vi "Stop All Helper Loops.vi"(8 "error in (no error)":errorcluster) -> (0 "error out":errorcluster)   [LabVIEW 2020, in "Helper Loop.lvclass"]
doc: "すべてのヘルパーループを終了し、リソースを破棄します。"
uses:
  Helper Loop.lvclass
  Helper Loop.lvclass/Helper Loop.ctl
  Sub/Helper Loop Map FGV Action.ctl
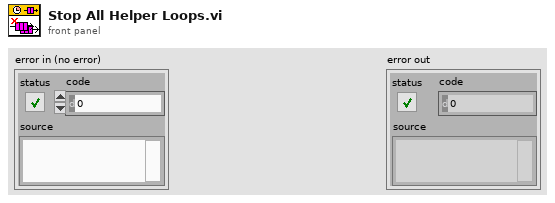
[diagram p1: front panel]
types:
  T1 = typedef "Helper Loop.lvclass/Helper Loop Map FGV Action.ctl" = enum16{"Get Pausing Helper Loop", "Register Active Helper Loop", "Pause Helper Loop", "Close Helper Loop", "Get All Helper Loops"}
  T2 = cluster{"Helper Loop Out":refnum<class "Helper Loop.lvclass">, "VI Reference":refnum<vi>}[]
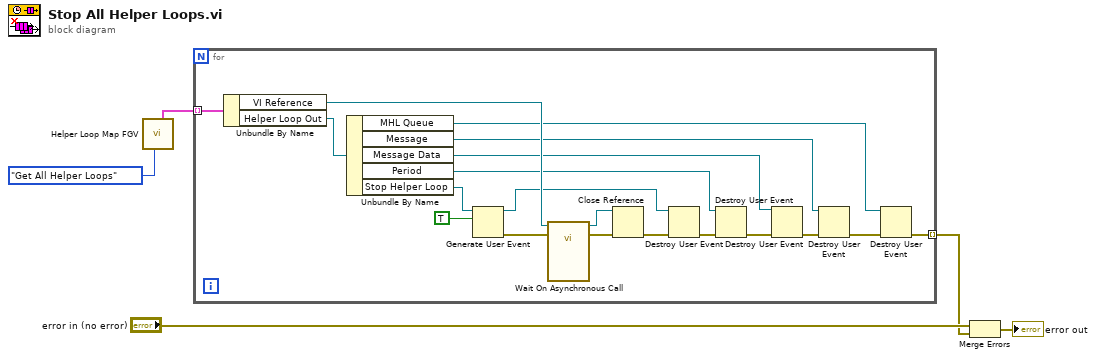
[diagram p0: block diagram]
diagram:
  n1 = call "Helper Loop Map FGV.vi"("Action"=Helper_Loop_Map_FGV_Action."Get All Helper Loops") -> ("All Helper Queues"=w4:T2)  [unwired: 7 in, 3 out]
  n2 = for {
    tunnel: w4 -> [w24] mode=indexing
    tunnel: [w6] -> w1 mode=indexing
    n3 = Unbundle By Name(w24) -> ("VI Reference"=w19:refnum<vi>, "Helper Loop Out"=w23:refnum<class "Helper Loop.lvclass">)
    n4 = Unbundle By Name(w23) -> ("MHL Queue"=w7:refnum<user-event>, "Message"=w8:refnum<user-event>, "Message Data"=w9:refnum<user-event>, "Period"=w10:refnum<user-event>, "Stop Helper Loop"=w22:refnum<user-event>)
    n5 = Generate User Event(user event=w22, event data cluster=TRUE ("event data")) -> (user event out=w15:refnum<user-event>, error out=w20:errorcluster)  [unwired: 2 in]
    n6 = call-by-ref "Wait On Asynchronous Call"(reference=w19, error in=w20) -> (reference out=w17:refnum<vi>, error out=w18:errorcluster)  [unwired: 11 in, 1 out]
    n7 = Close Reference(reference=w17, error in (no error)=w18) -> (error out=w16:errorcluster)
    n8 = Destroy User Event(user event=w15, error in=w16) -> (error out=w14:errorcluster)
    n9 = Destroy User Event(user event=w10, error in=w14) -> (error out=w13:errorcluster)
    n10 = Destroy User Event(user event=w9, error in=w13) -> (error out=w12:errorcluster)
    n11 = Destroy User Event(user event=w8, error in=w12) -> (error out=w11:errorcluster)
    n12 = Destroy User Event(user event=w7, error in=w11) -> (error out=w6:errorcluster)
  }
  n13 = Merge Errors("error in (no error)", w1) -> (→"error out":errorcluster)
